vi "Sous_VI_Sceaux.vi"() -> ()   [LabVIEW 2017]
uses:
  enum_bras.ctl
panel:
  out "Numérique 3":dbl
  out "Numérique 2":dbl
  out "Numérique":dbl
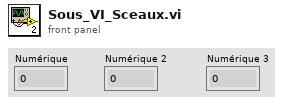
[diagram p1: front panel]
types:
  T1 = typedef "enum_bras.ctl" = enum16{"Depart Bras", "Clapet Bras", "Inactif Bras", "Seaux Bras"}
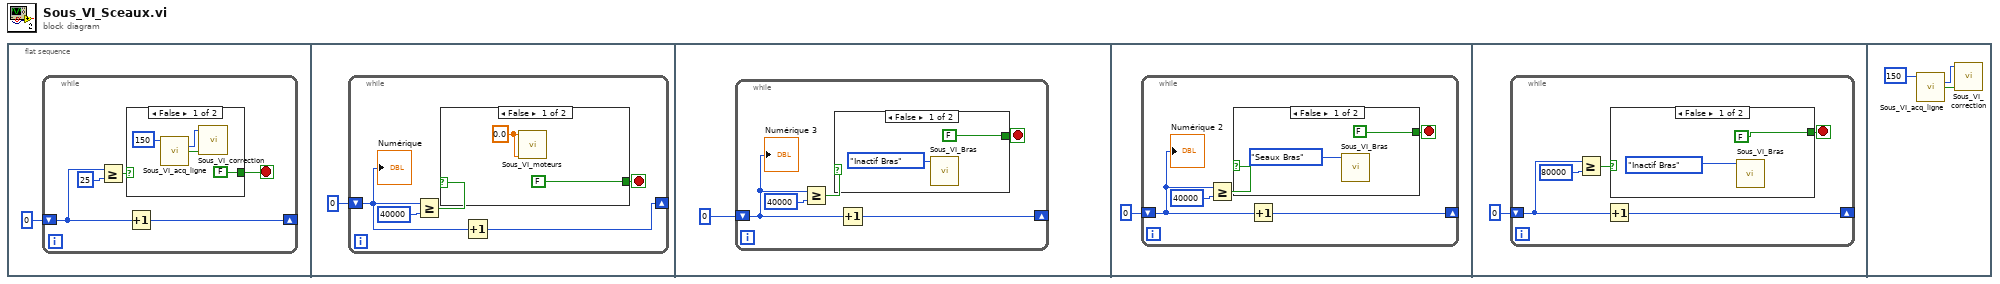
[diagram p0: block diagram]
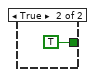
[diagram p2: hidden frame]
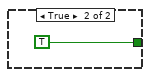
[diagram p3: hidden frame]
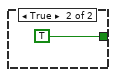
[diagram p4: hidden frame]
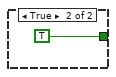
[diagram p5: hidden frame]
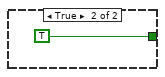
[diagram p6: hidden frame]
diagram:
  n1 = flat-sequence {
    frame #0 {
      n2 = while {
        shift-right: [w6] -> _
        shift-left: 0 -> [w3]
        stop <- w4 stop-if-true
        n3 = Greater Or Equal?(x=w3, y=25) -> (x >= y?=w5:bool)
        n4 = case shown="False" w5 {
          tunnel: [FALSE TRUE] -> w4
          frame False {
            n5 = call "Sous_VI_acq_ligne.vi"("Seuil"=150) -> ("Décalage"=w9:u32, "G/D ?"=w8:bool)  [unwired: 10 in, 3 out]
            n6 = call "Sous_VI_correction.vi"("G/D ?"=w8, "Décalage"=w9) -> ()  [unwired: 10 in]
          }
          frame True {
          }
        }
        n7 = Increment(x=w3) -> (x+1=w6:i32)
      }
    }
    frame #1 {
      n8 = while {
        shift-right: [w17] -> _
        shift-left: 0 -> [w13]
        stop <- w15 stop-if-true
        n9 = Greater Or Equal?(x=w13, y=40000) -> (x >= y?=w16:bool)
        n10 = case shown="False" w16 {
          tunnel: [FALSE TRUE] -> w15
          frame False {
            w18 = 0.0 ("Moteur Gauche")
            n11 = call "Sous_VI_moteurs.vi"("Moteur Droit"=w18, "Moteur Gauche"=w18) -> ()  [unwired: 10 in]
          }
          frame True {
          }
        }
        n12 = Increment(x=w13) -> (x+1=w17:i32)
        "Numérique" <- w13
      }
    }
    frame #2 {
      n13 = while {
        shift-right: [w26] -> _
        shift-left: 0 -> [w22]
        stop <- w24 stop-if-true
        n14 = Greater Or Equal?(x=w22, y=40000) -> (x >= y?=w25:bool)
        n15 = case shown="False" w25 {
          tunnel: [FALSE TRUE] -> w24
          frame False {
            n16 = call "Sous_VI_Bras.vi"("Enum bras"=enum_bras."Inactif Bras") -> ()  [unwired: 11 in]
          }
          frame True {
          }
        }
        n17 = Increment(x=w22) -> (x+1=w26:i32)
        "Numérique 3" <- w22
      }
    }
    frame #3 {
      n18 = while {
        shift-right: [w35] -> _
        shift-left: 0 -> [w31]
        stop <- w33 stop-if-true
        n19 = Greater Or Equal?(x=w31, y=40000) -> (x >= y?=w34:bool)
        n20 = case shown="False" w34 {
          tunnel: [FALSE TRUE] -> w33
          frame False {
            n21 = call "Sous_VI_Bras.vi"("Enum bras"=enum_bras."Seaux Bras") -> ()  [unwired: 11 in]
          }
          frame True {
          }
        }
        n22 = Increment(x=w31) -> (x+1=w35:i32)
        "Numérique 2" <- w31
      }
    }
    frame #4 {
      n23 = while {
        shift-right: [w44] -> _
        shift-left: 0 -> [w40]
        stop <- w42 stop-if-true
        n24 = Greater Or Equal?(x=w40, y=80000) -> (x >= y?=w43:bool)
        n25 = Increment(x=w40) -> (x+1=w44:i32)
        n26 = case shown="False" w43 {
          tunnel: [FALSE TRUE] -> w42
          frame False {
            n27 = call "Sous_VI_Bras.vi"("Enum bras"=enum_bras."Inactif Bras") -> ()  [unwired: 11 in]
          }
          frame True {
          }
        }
      }
    }
    frame #5 {
      n28 = call "Sous_VI_acq_ligne.vi"("Seuil"=150) -> ("Décalage"=w50:u32, "G/D ?"=w49:bool)  [unwired: 10 in, 3 out]
      n29 = call "Sous_VI_correction.vi"("G/D ?"=w49, "Décalage"=w50) -> ()  [unwired: 10 in]
    }
  }
